vi "Valve pilot lamp.vi"(0 "Position word":u32, 1 "Bit offset":u32, 2 "Physical selectors":u32, 3 "Selector quality":u32) -> (15 "Lamp":picture)   [LabVIEW 2025]
doc: "Render the live valve state. Grey means unavailable or invalid."
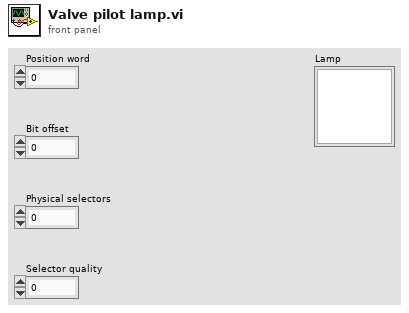
[diagram p1: front panel]
types:
  T1 = cluster{"left":i16, "top":i16, "right":i16, "bottom":i16}
  T2 = cluster{"left":i16, "top":i16, "right":i16, "bottom":i16}[]
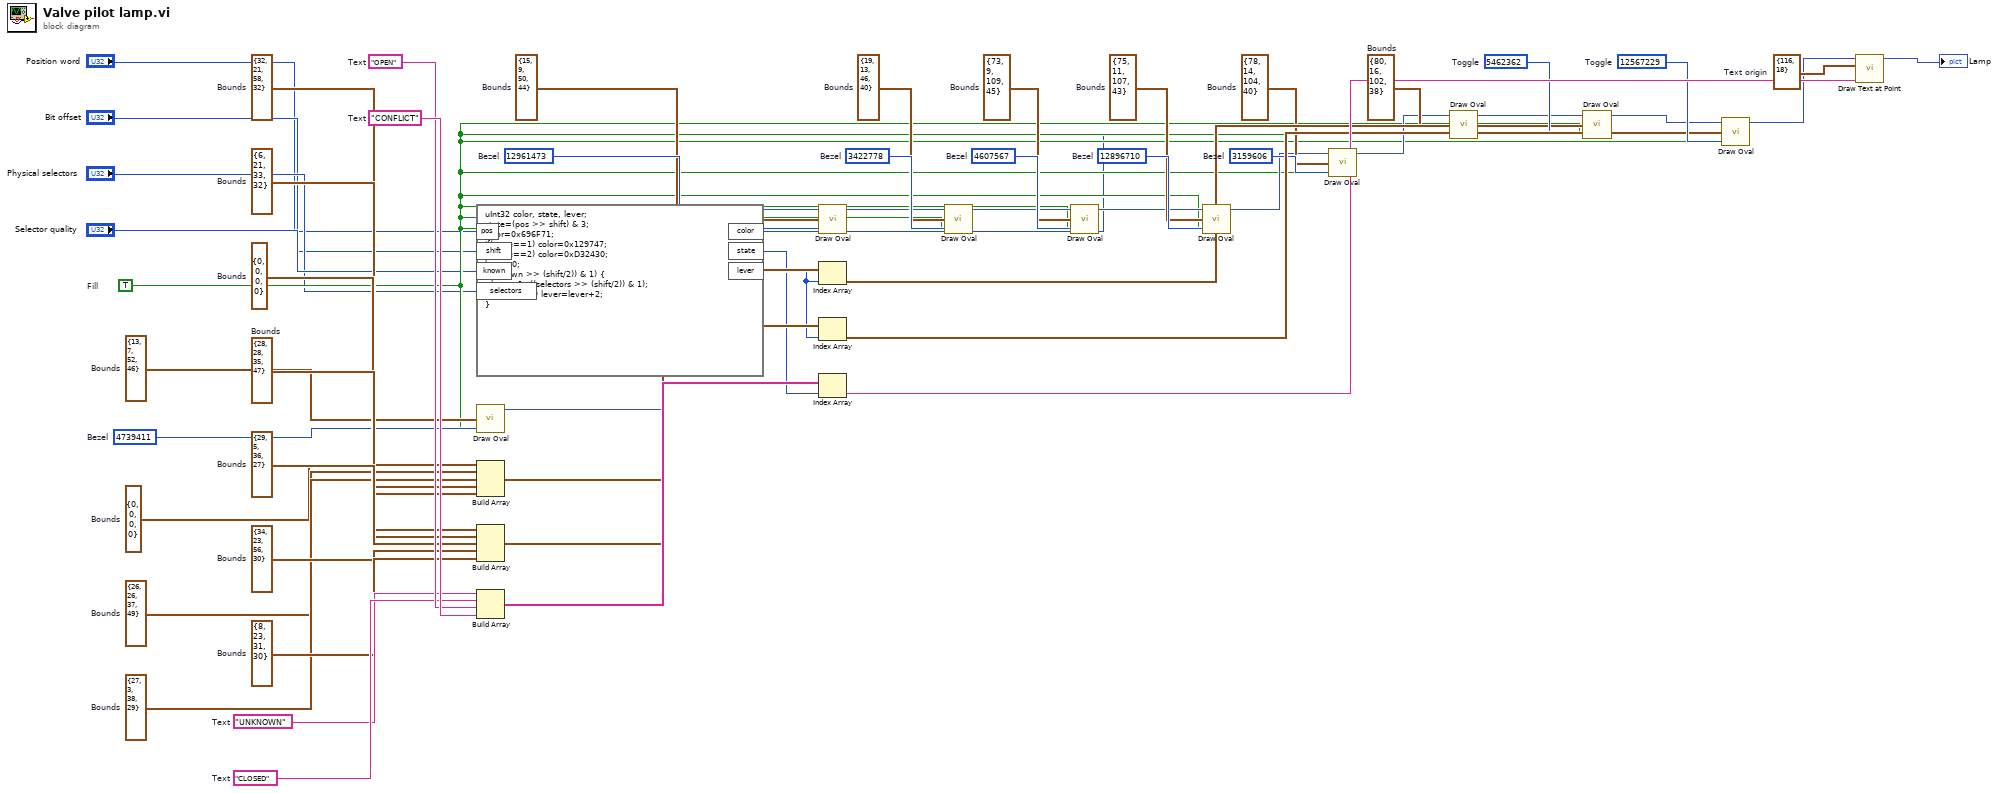
[diagram p0: block diagram]
diagram:
  w53 = cluster{"x":i16, "y":i16} {"x"=116, "y"=18}  # Text origin
  w50 = "CONFLICT"  # Text
  w49 = "OPEN"  # Text
  w48 = "CLOSED"  # Text
  w47 = "UNKNOWN"  # Text
  w45 = u32 12567229  # Toggle
  w42 = T1 {"left"=8, "top"=23, "right"=31, "bottom"=30}  # Bounds
  w41 = T1 {"left"=34, "top"=23, "right"=56, "bottom"=30}  # Bounds
  w40 = T1 {"left"=29, "top"=5, "right"=36, "bottom"=27}  # Bounds
  w39 = T1 {"left"=28, "top"=28, "right"=35, "bottom"=47}  # Bounds
  w38 = T1 {"left"=0, "top"=0, "right"=0, "bottom"=0}  # Bounds
  w36 = u32 5462362  # Toggle
  w33 = T1 {"left"=6, "top"=21, "right"=33, "bottom"=32}  # Bounds
  w32 = T1 {"left"=32, "top"=21, "right"=58, "bottom"=32}  # Bounds
  w31 = T1 {"left"=27, "top"=3, "right"=38, "bottom"=29}  # Bounds
  w30 = T1 {"left"=26, "top"=26, "right"=37, "bottom"=49}  # Bounds
  w29 = T1 {"left"=0, "top"=0, "right"=0, "bottom"=0}  # Bounds
  w27 = T1 {"left"=80, "top"=16, "right"=102, "bottom"=38}  # Bounds
  w25 = u32 3159606  # Bezel
  w24 = T1 {"left"=78, "top"=14, "right"=104, "bottom"=40}  # Bounds
  w22 = u32 12896710  # Bezel
  w21 = T1 {"left"=75, "top"=11, "right"=107, "bottom"=43}  # Bounds
  w19 = u32 4607567  # Bezel
  w18 = T1 {"left"=73, "top"=9, "right"=109, "bottom"=45}  # Bounds
  w16 = u32 3422778  # Bezel
  w15 = T1 {"left"=19, "top"=13, "right"=46, "bottom"=40}  # Bounds
  w13 = u32 12961473  # Bezel
  w12 = T1 {"left"=15, "top"=9, "right"=50, "bottom"=44}  # Bounds
  w10 = u32 4739411  # Bezel
  w9 = T1 {"left"=13, "top"=7, "right"=52, "bottom"=46}  # Bounds
  w8 = TRUE  # Fill
  n1 = formula code="uInt32 color, state, lever;\nstate=(pos >> shift) & 3;\ncolor=0x696F71;\nif(state==1) color=0x129747;\nif(state==2) color=0xD32430;\nlever=0;\nif((known >> (shift/2)) & 1) {\n  lever=1+((selectors >> (shift/2)) & 1);\n  if(shift==6) lever=lever+2;\n}"("pos"="Position word", "shift"="Bit offset", "known"="Selector quality", "selectors"="Physical selectors") -> ("color"=w5:u32, "state"=w6:u32, "lever"=w7:u32)
  n2 = call <vilib>:"Draw Oval.vi"("rect"=w9, "fill?(F)"=w8, "color(black)"=w10) -> ("new picture"=w11:picture)  [unwired: 6 in]
  n3 = Build Array(w29, w30, w31, w32, w33) -> (w34:T2)
  n4 = Build Array(w38, w39, w40, w41, w42) -> (w43:T2)
  n5 = Build Array(w47, w48, w49, w50) -> (w51:string[])
  n6 = call <vilib>:"Draw Oval.vi"("picture"=w11, "rect"=w12, "fill?(F)"=w8, "color(black)"=w13) -> ("new picture"=w14:picture)  [unwired: 5 in]
  n7 = Index Array(array=w34, index=w7) -> (element=w35:T1)
  n8 = Index Array(array=w43, index=w7) -> (element=w44:T1)
  n9 = Index Array(array=w51, index=w6) -> (element=w52:string)
  n10 = call <vilib>:"Draw Oval.vi"("picture"=w14, "rect"=w15, "fill?(F)"=w8, "color(black)"=w16) -> ("new picture"=w17:picture)  [unwired: 5 in]
  n11 = call <vilib>:"Draw Oval.vi"("picture"=w17, "rect"=w18, "fill?(F)"=w8, "color(black)"=w19) -> ("new picture"=w20:picture)  [unwired: 5 in]
  n12 = call <vilib>:"Draw Oval.vi"("picture"=w20, "rect"=w21, "fill?(F)"=w8, "color(black)"=w22) -> ("new picture"=w23:picture)  [unwired: 5 in]
  n13 = call <vilib>:"Draw Oval.vi"("picture"=w23, "rect"=w24, "fill?(F)"=w8, "color(black)"=w25) -> ("new picture"=w26:picture)  [unwired: 5 in]
  n14 = call <vilib>:"Draw Oval.vi"("picture"=w26, "rect"=w27, "fill?(F)"=w8, "color(black)"=w5) -> ("new picture"=w28:picture)  [unwired: 5 in]
  n15 = call <vilib>:"Draw Oval.vi"("picture"=w28, "rect"=w35, "fill?(F)"=w8, "color(black)"=w36) -> ("new picture"=w37:picture)  [unwired: 5 in]
  n16 = call <vilib>:"Draw Oval.vi"("picture"=w37, "rect"=w44, "fill?(F)"=w8, "color(black)"=w45) -> ("new picture"=w46:picture)  [unwired: 5 in]
  n17 = call <vilib>:"Draw Text at Point.vi"("text"=w52, "origin"=w53, "picture"=w46) -> ("new picture"=→"Lamp":picture)  [unwired: 7 in, 1 out]
